vi "Start Sequence.vi"(8 "error in":errorcluster, 11 "Sequence Executor in":refnum<class "Sequence Executor.lvclass">) -> (0 "error out":errorcluster, 3 "Sequence Executor out":refnum<class "Sequence Executor.lvclass">)   [LabVIEW 2026, in "Sequence Executor.lvclass"]
doc: "Starts the loaded sequence: refuses (Status only, no error) unless Loaded and not Running. Resets Results, Step Index 0, Running T, Overall Verdict empty, Phase Idle, Status RUNNING, then Begin Step. Message: Start Sequence Msg (no payload)."
uses:
  Sequence Executor.lvclass
  Sequence Executor.lvclass/Sequence Executor.ctl
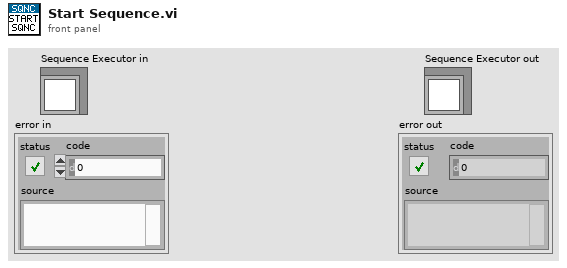
[diagram p1: front panel]
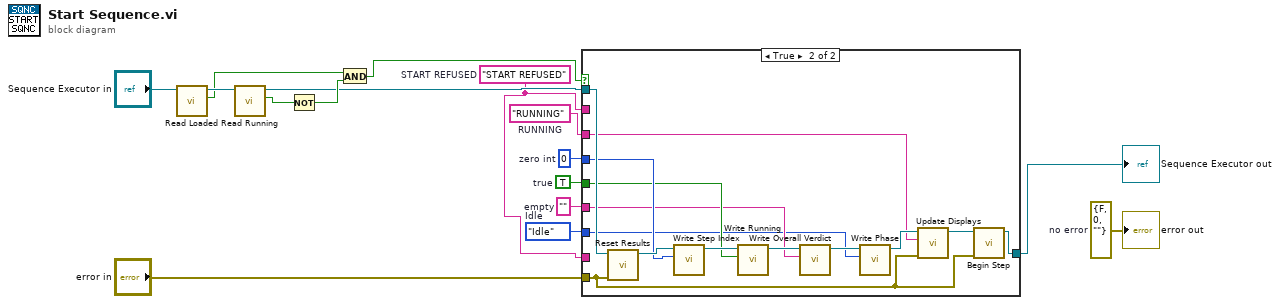
[diagram p0: block diagram]
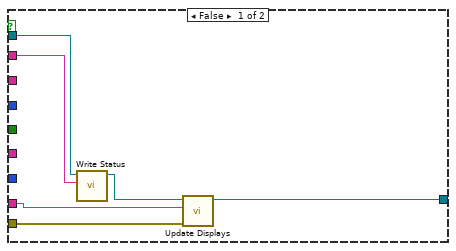
[diagram p2: hidden frame]
diagram:
  w9 = "START REFUSED"  # START REFUSED
  w4 = "RUNNING"  # RUNNING
  w5 = enum16{"Idle", "Settling", "Dwell", "Complete"}."Idle"  # Idle
  w6 = ""  # empty
  w8 = 0  # zero int
  w7 = TRUE  # true
  w1 = errorcluster {"status"=FALSE, "code"=0, "source"=""}  # no error
  n1 = call "Read Loaded.vi"("Sequence Executor in"="Sequence Executor in") -> ("Loaded"=w13:bool, "Sequence Executor out"=w15:refnum<class "Sequence Executor.lvclass">)  [unwired: 8 in, 1 out]
  n2 = call "Read Running.vi"("Sequence Executor in"=w15) -> ("Running"=w14:bool, "Sequence Executor out"=w11:refnum<class "Sequence Executor.lvclass">)  [unwired: 8 in, 1 out]
  n3 = Not(x=w14) -> (.not. x?=w12:bool)
  n4 = And(x=w13, y=w12) -> (x .and. y?=w3:bool)
  n5 = case shown="True" w3 {
    tunnel: w11 -> [w22 w36]
    tunnel: "error in" -> [w18 w24]
    tunnel: w9 -> [w21 _]
    tunnel: w9 -> [w19 _]
    tunnel: [w17 w23] -> w2
    tunnel: w8 -> [_ w34]
    tunnel: w7 -> [_ w32]
    tunnel: w6 -> [_ w30]
    tunnel: w5 -> [_ w28]
    tunnel: w4 -> [_ w26]
    frame False {
      n6 = call "Write Status.vi"("Status"=w21, "Sequence Executor in"=w22) -> ("Sequence Executor out"=w20:refnum<class "Sequence Executor.lvclass">)  [unwired: 8 in, 1 out]
      n7 = call "Update Displays.vi"("error in"=w18, "Status"=w19, "Sequence Executor in"=w20) -> ("Sequence Executor out"=w17:refnum<class "Sequence Executor.lvclass">)  [unwired: 7 in, 1 out]
    }
    frame True {
      n8 = call "Reset Results.vi"("error in"=w24, "Sequence Executor in"=w36) -> ("Sequence Executor out"=w35:refnum<class "Sequence Executor.lvclass">)  [unwired: 8 in, 1 out]
      n9 = call "Write Step Index.vi"("Step Index"=w34, "Sequence Executor in"=w35) -> ("Sequence Executor out"=w33:refnum<class "Sequence Executor.lvclass">)  [unwired: 8 in, 1 out]
      n10 = call "Write Running.vi"("Running"=w32, "Sequence Executor in"=w33) -> ("Sequence Executor out"=w31:refnum<class "Sequence Executor.lvclass">)  [unwired: 8 in, 1 out]
      n11 = call "Write Overall Verdict.vi"("Overall Verdict"=w30, "Sequence Executor in"=w31) -> ("Sequence Executor out"=w29:refnum<class "Sequence Executor.lvclass">)  [unwired: 8 in, 1 out]
      n12 = call "Write Phase.vi"("Step Phase"=w28, "Sequence Executor in"=w29) -> ("Sequence Executor out"=w27:refnum<class "Sequence Executor.lvclass">)  [unwired: 8 in, 1 out]
      n13 = call "Update Displays.vi"("error in"=w24, "Status"=w26, "Sequence Executor in"=w27) -> ("Sequence Executor out"=w25:refnum<class "Sequence Executor.lvclass">)  [unwired: 7 in, 1 out]
      n14 = call "Begin Step.vi"("error in"=w24, "Sequence Executor in"=w25) -> ("Sequence Executor out"=w23:refnum<class "Sequence Executor.lvclass">)  [unwired: 8 in, 1 out]
    }
  }
  "Sequence Executor out" <- w2
  "error out" <- w1
